vi "Target Environment To Number.vi"(11 "Target (Process)":T1 items=["Process", "User", "Machine"]) -> (3 "Numeric Value":i32)   [LabVIEW 2019, in "SLL Environment Variable.lvlib"]
doc: "Convert <B>Target</B> environment enum to equivalent <B>Numeric Value</B>."
uses:
  SLL Environment Variable.lvlib
  _Typedef/Target Environment Enum.ctl
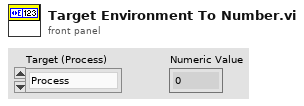
[diagram p1: front panel]
types:
  T1 = typedef "SLL Environment Variable.lvlib/Target Environment Enum.ctl" = i32
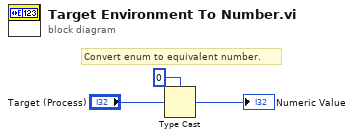
[diagram p0: block diagram]
diagram:
  # "Convert enum to equivalent number."
  n1 = Type Cast(type=0, x="Target (Process)") -> (*(type *) &x=→"Numeric Value":i32)
